vi "Init with Value.vi"(8 "error in":errorcluster, 10 "Value":variant, 11 "Image in":refnum<class "Image.lvclass">) -> (0 "error out":errorcluster, 3 "Image out":refnum<class "Image.lvclass">)   [LabVIEW 2020, in "SourceGrid.lvlib" / "Image.lvclass"]
uses:
  Image.lvclass
  System.Drawing
  D:/git/Sourcegrid-LabVIEW/source/SourceGrid.dll
  SourceGrid.dll
  Image.lvclass/Image.ctl
  Cell/Cell.lvclass
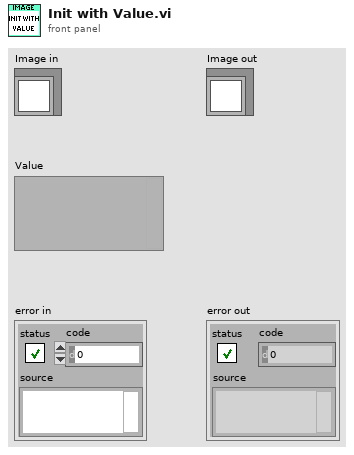
[diagram p1: front panel]
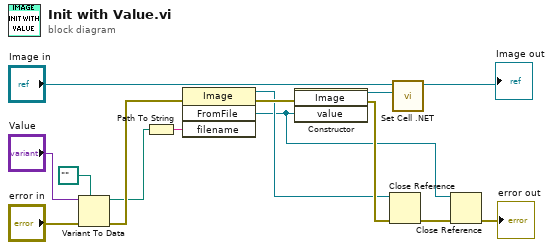
[diagram p0: block diagram]
diagram:
  n1 = Variant To Data(error in="error in", type=path "", Variant="Value") -> (data=w4:path, error out=w7:errorcluster)
  n2 = Path To String(path=w4) -> (string=w8:string)
  n3 = invoke class="Image" method="FromFile"(error in=w7, "filename"=w8) -> (reference out=w9:refnum<k24>, error out=w10:errorcluster, "FromFile"=w1:refnum<k24>)  [unwired: 2 in, 1 out]
  n4 = constructor class="Image"(error in=w10, "value"=w1) -> (reference out=w3:refnum<k24>, error out=w15:errorcluster)  [unwired: 2 in, 2 out]
  n5 = Close Reference(reference=w9, error in (no error)=w15) -> (error out=w13:errorcluster)
  n6 = call "Set Cell .NET.vi"("Cell .NET"=w3, "Cell in"="Image in") -> ("Cell out"=→"Image out":refnum<class "Image.lvclass">)  [unwired: 9 in]
  n7 = Close Reference(reference=w1, error in (no error)=w13) -> (error out=→"error out":errorcluster)
